vi "KYFG Set Grabber Value Int.vi"(8 "error in (no error)":errorcluster, 9 "value":i64, 10 "paramName":string, 11 "camHandle":u32) -> (0 "error out":errorcluster, 3 "camHandle out":u32)   [LabVIEW 2023, in "KYFGLib_lv.lvlib"]
doc: "KYFG_API FGSTATUS KYFG_SetCameraValueEnum_ByValueName(CAMHANDLE camHandle, const char *paramName, const char *paramValueName);"
uses:
  KYFGLib_lv.lvlib
  KYFGLib.dll
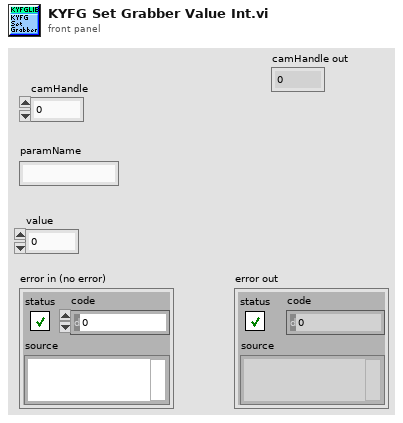
[diagram p1: front panel]
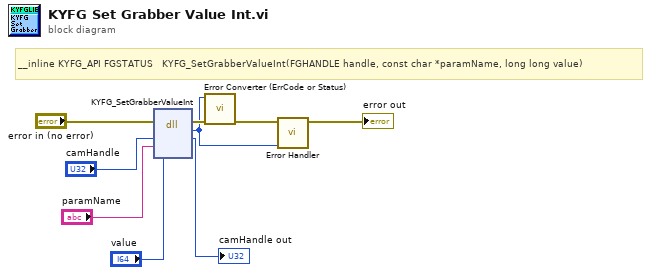
[diagram p0: block diagram]
diagram:
  # "__inline KYFG_API FGSTATUS   KYFG_SetGrabberValueInt(FGHANDLE handle, const char *paramName, long long value)"
  n1 = dll-call lib="KYFGLib.dll" fn="KYFG_SetGrabberValueInt"(error in="error in (no error)", "camHandle"="camHandle", "paramName"="paramName", "value"="value") -> (error out=w6:errorcluster, "return type"=w3:u32, "camHandle"=→"camHandle out":u32)  [unwired: 4 in, 1 out]
  n2 = call "Error Converter (ErrCode or Status).vi"("error in (no error)"=w6, "error code"=w3) -> ("error out"=w5:errorcluster)  [unwired: 9 in]
  n3 = call "Error Handler.vi"("Return Code"=w3, "Error In"=w5) -> ("Error Out"=→"error out":errorcluster)  [unwired: 9 in]
